vi "4bar setpoint and immediate.vi"(4 "Cargo Ship for Cargo":dbl, 5 "Cargo Ship for Hatch":dbl, 6 "Operator X Button":bool, 7 "Hatch Setpoint":dbl, 8 "Operator Y Button":bool, 9 "Operator B Button":bool, 10 "Operator A Button":bool, 11 "Operator Right Joystick Y in":dbl) -> (3 "Output":cluster{"Control Mode":T1, "Output":dbl} {"Control Mode" items=["PercentOutput"=0, "Position"=1, "Velocity"=2, "Current"=3, "Follower"=5, "MotionProfile"=6, "MotionMagic"=7, "MotionProfileArc"=10, "Disabled"=15]})   [LabVIEW 2018]
uses:
  <vilib>/Rock Robotics/WPI/ThirdParty/Phoenix-LabVIEW/Motor Controller/Controls/CTRE_Phoenix_MotorControl_ControlMode.ctl
  4barCommands.ctl
  Infrastructure/Constants.vi
  Robot Global Data.vi
  <vilib>/Rock Robotics/Network Tables/NT Write Number.vi
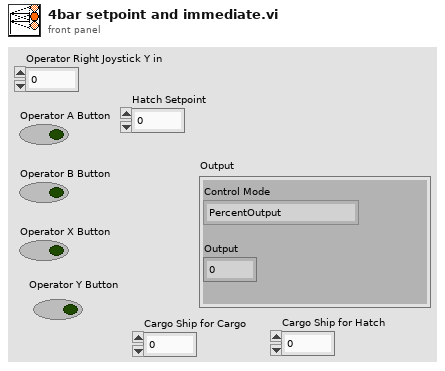
[diagram p1: front panel]
types:
  T1 = typedef "CTRE_Phoenix_MotorControl_ControlMode.ctl" = u16
  T2 = typedef "4barCommands.ctl" = enum16{"Immediate", "Hold", "Setpoint"}
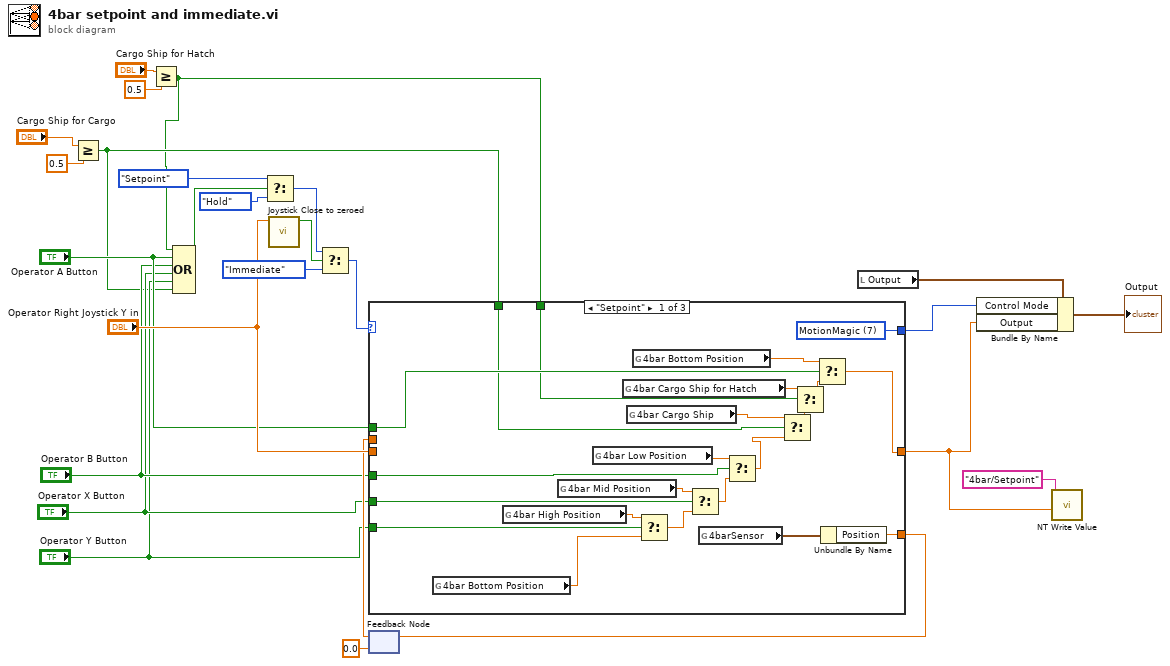
[diagram p0: block diagram]
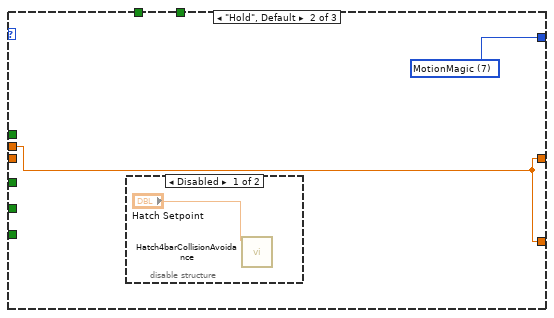
[diagram p2: hidden frame]
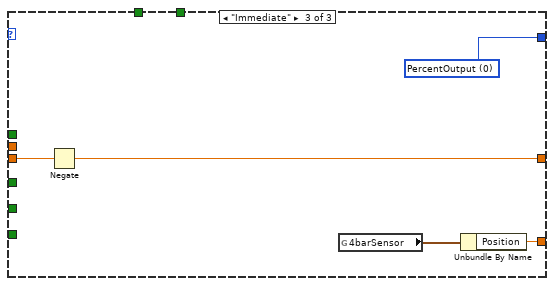
[diagram p4: hidden frame]
diagram:
  n1 = Greater Or Equal?(x="Cargo Ship for Cargo", y=0.5 ("Position")) -> (x >= y?=w4:bool)
  n2 = Greater Or Equal?(x="Cargo Ship for Hatch", y=0.5 ("Position")) -> (x >= y?=w1:bool)
  n3 = Compound Arithmetic op=OR(w1, "Operator A Button", "Operator B Button", "Operator X Button", "Operator Y Button", w4) -> (w11:bool)
  n4 = Select(t=4barCommands."Setpoint", s=w11, f=4barCommands."Hold" ("t")) -> (s? t:f=w20:T2)
  n5 = call "Joystick Close to zeroed.vi"("Joystick"="Operator Right Joystick Y in") -> ("=0?"=w18:bool)  [unwired: 10 in]
  n6 = Select(t=w20, s=w18, f=4barCommands."Immediate") -> (s? t:f=w25:T2)
  n7 = feedback #1(0.0 ("Position")) -> (w21:dbl)
  n8 = case shown="\"Setpoint\"" w25 {
    tunnel: "Operator X Button" -> [w45 _ _]
    tunnel: "Operator B Button" -> [w32 _ _]
    tunnel: "Operator A Button" -> [w44 _ _]
    tunnel: "Operator Right Joystick Y in" -> [_ _ w55]
    tunnel: [w43 w50 w56] -> w22
    tunnel: [w31 w49 w54] -> w7
    tunnel: "Operator Y Button" -> [w41 _ _]
    tunnel: w21 -> [_ w49 _]
    tunnel: [w38 w49 w52] -> w10
    tunnel: w4 -> [w33 _ _]
    tunnel: w1 -> [w29 _ _]
    frame "Setpoint" {
      w43 = T1 7 items=["PercentOutput"=0, "Position"=1, "Velocity"=2, "Current"=3, "Follower"=5, "MotionProfile"=6, "MotionMagic"=7, "MotionProfileArc"=10, "Disabled"=15] ("Control Mode")
      n9 = global read "Constants.vi" "4bar Bottom Position"() -> (w37:dbl)
      n10 = global read "Constants.vi" "4bar High Position"() -> (w42:dbl)
      n11 = global read "Constants.vi" "4bar Mid Position"() -> (w48:dbl)
      n12 = global read "Constants.vi" "4bar Low Position"() -> (w36:dbl)
      n13 = global read "Constants.vi" "4bar Cargo Ship for Hatch"() -> (w30:dbl)
      n14 = global read "Constants.vi" "4bar Cargo Ship"() -> (w47:dbl)
      n15 = global read "Constants.vi" "4bar Bottom Position"() -> (w46:dbl)
      n16 = Select(t=w42, s=w41, f=w37) -> (s? t:f=w40:dbl)
      n17 = Select(t=w48, s=w45, f=w40) -> (s? t:f=w35:dbl)
      n18 = global read "Robot Global Data.vi" "4barSensor"() -> (w39:cluster{"Position":dbl, "Velocity":dbl})
      n19 = Select(t=w36, s=w32, f=w35) -> (s? t:f=w34:dbl)
      n20 = Select(t=w47, s=w33, f=w34) -> (s? t:f=w27:dbl)
      n21 = Select(t=w30, s=w29, f=w27) -> (s? t:f=w28:dbl)
      n22 = Select(t=w46, s=w44, f=w28) -> (s? t:f=w31:dbl)
      n23 = Unbundle By Name(w39) -> ("Position"=w38:dbl)
    }
    frame "Hold", Default {
      w50 = T1 7 items=["PercentOutput"=0, "Position"=1, "Velocity"=2, "Current"=3, "Follower"=5, "MotionProfile"=6, "MotionMagic"=7, "MotionProfileArc"=10, "Disabled"=15] ("Control Mode")
      n24 = disable-structure shown="Disabled" {
        frame Disabled {
          n25 = call "Hatch4barCollisionAvoidance.vi"("Hatch Setpoint"="Hatch Setpoint") -> ()  [unwired: 10 in, 1 out]
        }
        frame Enabled {
        }
      }
    }
    frame "Immediate" {
      w56 = T1 0 items=["PercentOutput"=0, "Position"=1, "Velocity"=2, "Current"=3, "Follower"=5, "MotionProfile"=6, "MotionMagic"=7, "MotionProfileArc"=10, "Disabled"=15] ("Control Mode")
      n26 = Negate(x=w55) -> (-x=w54:dbl)
      n27 = global read "Robot Global Data.vi" "4barSensor"() -> (w53:cluster{"Position":dbl, "Velocity":dbl})
      n28 = Unbundle By Name(w53) -> ("Position"=w52:dbl)
    }
  }
  n29 = feedback-in #1(w10) -> ()
  n30 = local read "Output"() -> (w23:cluster{"Control Mode":T1, "Output":dbl})
  n31 = Bundle By Name(cluster=w23, "Control Mode"=w22, "Output"=w7) -> (→"Output":cluster{"Control Mode":T1, "Output":dbl})
  n32 = call-poly <vilib>:"NT Write Value.vi"("Numeric"=w7, "Name"="4bar/Setpoint") -> ()  [unwired: 9 in, 1 out]
